vi "Test RUN EPC.vi"(2 "Adresse régulateur":u8, 3 "Port COM run 1 REG":refnum<visa-resource-name>) -> (0 "Adresse régulateur 2":u8, 1 "En RUN":bool)   [LabVIEW 2022 SP3]
uses:
  Variables globales/Variables glob EUROTHERM.vi
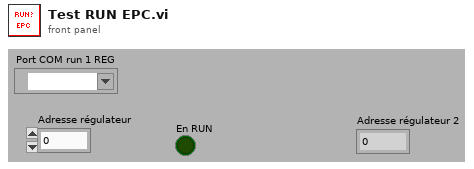
[diagram p1: front panel]
types:
  T1 = typedef "Semaphore RefNum" = refnum<k1>
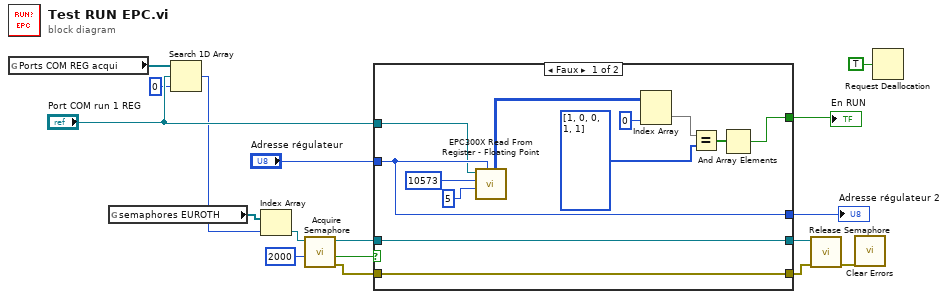
[diagram p0: block diagram]
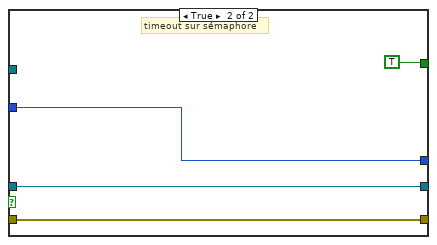
[diagram p2: hidden frame]
diagram:
  n1 = global read "Variables glob EUROTHERM.vi" "Ports COM REG acqui"() -> (w4:refnum<visa-resource-name>[])
  n2 = global read "Variables glob EUROTHERM.vi" "semaphores EUROTH"() -> (w6:T1[])
  n3 = Search 1D Array(1D array=w4, element="Port COM run 1 REG", start index (0)=0 ("indice de départ (0)")) -> (index of element=w1:i32)
  n4 = Index Array(array=w6, index=w1) -> (element=w5:T1)
  n5 = call <vilib>:"Acquire Semaphore.vi"("ms timeout (-1)"=2000, "semaphore"=w5) -> ("error out"=w10:errorcluster, "timed out"=w12:bool, "semaphore out"=w11:T1)  [unwired: 3 in]
  n6 = case shown="Faux" w12 {
    tunnel: "Adresse régulateur" -> [w24 w31]
    tunnel: [w24 w31] -> w15
    tunnel: [w25 TRUE] -> w14
    tunnel: w11 -> [w29 w32]
    tunnel: w10 -> [w28 w33]
    tunnel: [w29 w32] -> w9
    tunnel: [w28 w33] -> w8
    tunnel: "Port COM run 1 REG" -> [w23 _]
    frame False {
      n7 = call "EPC300X Read From Register - Floating Point.vi"("Unit Address (1)"=w24, "Num Of Reg (1)"=u16 5, "Register Address (0)"=u16 10573, "VISA session"=w23) -> ("Data 2 (U16)"=w26:u16[][])  [unwired: 2 in, 5 out]
      n8 = Index Array(array=w26, index (col)=0 ("indice désactivé (col)")) -> (element=w20:u16[])  [unwired: 1 in]
      n9 = Equal?(x=w20, y=u16[] [1, 0, 0, 1, 1]) -> (x = y?=w18:bool[])
      n10 = And Array Elements(Boolean array=w18) -> (logical AND=w25:bool)
    }
    frame True {
      # "timeout sur sémaphore"
    }
  }
  "Adresse régulateur 2" <- w15
  "En RUN" <- w14
  n11 = call <vilib>:"Release Semaphore.vi"("error in (no error)"=w8, "semaphore"=w9) -> ("error out"=w7:errorcluster)  [unwired: 4 in, 1 out]
  n12 = call <vilib>:"Clear Errors.vi"("error in (no error)"=w7) -> ()  [unwired: 5 in, 2 out]
  n13 = Request Deallocation(TRUE ("flag")) -> ()
